vi "MovCorrFuncs 0.1.vi"(7 "Boundary":dbl, 8 "error in (no error)":errorcluster, 9 "MovCorrFunc":T5(ring), 10 "LUT1":cluster{u16, u16}(slide)={0, 4095} caption="Slide" scale=0.0..4095.0, 11 "Image":T3(plugin-control)) -> (0 "error out":errorcluster, 2 "Reference Rectangles":i16[][](array[numeric]), 3 "Reference Screen":T3(plugin-control))   [LabVIEW 2020]
uses:
  <vilib>/vision/Image Controls.llb/IMAQ Image.ctl
panel:
  in  "LUT 2":cluster{i16, i16}(slide)={0, 4095} scale=0.0..4095.0
  in  "LUT":cluster{i16, i16}(slide)={0, 4095} scale=0.0..4095.0
  out "Lines":T1(array[cluster]) {"End Point"."Y" format="%.2f"; "End Point"."X" format="%.2f"; "Start Point"."Y" format="%.2f"; "Start Point"."X" format="%.2f"}
  out "Number of Matches Returned":i32
  out "most Verital":T2
  out "most horizontal":T2
  out "got copy":bool=TRUE
  out "upper":u16
  out "lower":u16
  out "Number of Particles":i32
  out "Mean Value":sgl format="%.2f"
  out "Histogram Graph":T4 {"Incremental Value" format="%.2f"; "Starting Value" format="%.2f"}
  out "temp copy":T3
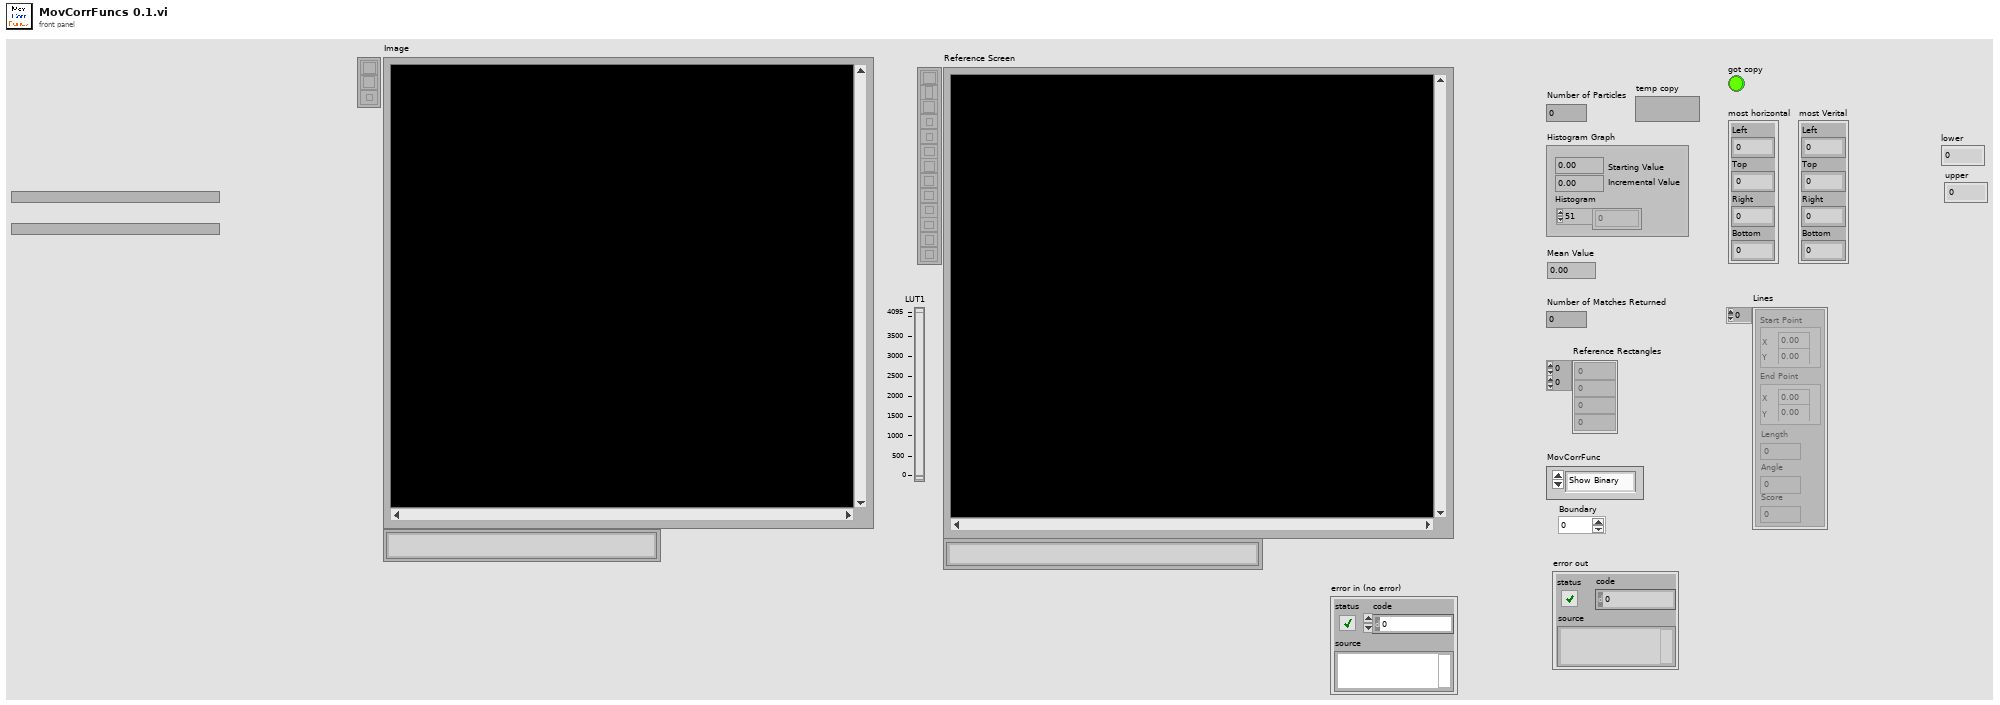
[diagram p1: front panel]
types:
  T1 = cluster{"Start Point":cluster{"X":sgl, "Y":sgl}, "End Point":cluster{"X":sgl, "Y":sgl}, "Length":dbl, "Angle":dbl, "Score":dbl}[]
  T2 = cluster{"Left":i32, "Top":i32, "Right":i32, "Bottom":i32}
  T3 = typedef "IMAQ Image.ctl" = refnum<image>
  T4 = cluster{"Starting Value":sgl, "Incremental Value":sgl, "Histogram":u32[]}
  T5 = enum16{"Show Binary", "Show Dendrite", "Find Lines"}
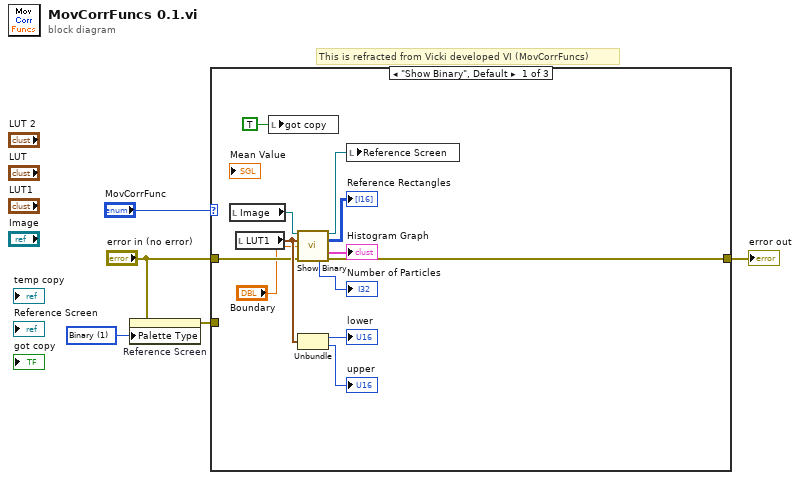
[diagram p0: block diagram]
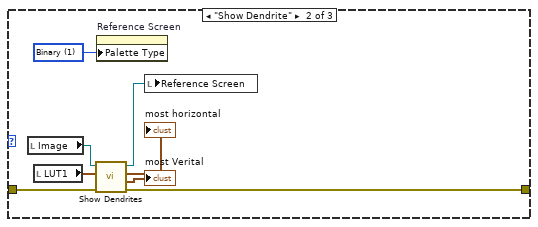
[diagram p2: hidden frame]
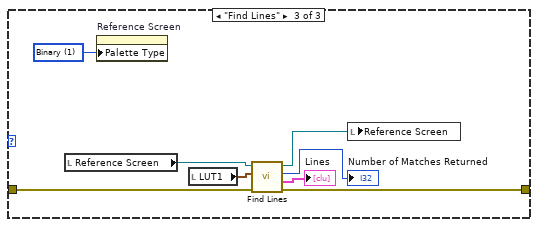
[diagram p3: hidden frame]
diagram:
  w3 = u32 1 items=["Grayscale", "Binary", "Gradient", "Rainbow", "Temperature", "User Defined"] ("Palette:Palette Type")
  # "This is refracted from Vicki developed VI (MovCorrFuncs)"
  n1 = property on="Reference Screen" class="ImageControl"(error in="error in (no error)", "Palette Type"=w3) -> (error out=w1:errorcluster)  [unwired: 1 in, 1 out]
  n2 = case shown="\"Show Binary\", Default" "MovCorrFunc" {
    tunnel: "error in (no error)" -> [w8 w20 w27]
    tunnel: [w7 w19 w26] -> w4
    tunnel: w1 -> [_ _ _]
    frame "Show Binary", Default {
      n3 = local read "Image"() -> (w12:T3)
      n4 = local read "LUT1"() -> (w9:cluster{u16, u16})
      n5 = local write "got copy"(TRUE) -> ()
      n6 = call "Show Binary.vi"("Input Image"=w12, "LUT1"=w9, "Boundary"="Boundary", "error in (no error)"=w8) -> ("Binary Image"=w10:T3, "Reference Rectangles"=→"Reference Rectangles":i16[][], "Histogram Graph"=→"Histogram Graph":T4, "Number of Particles"=→"Number of Particles":i32, "error out"=w7:errorcluster)  [unwired: 7 in]
      n7 = Unbundle(w9) -> (→"lower":u16, →"upper":u16)
      n8 = local write "Reference Screen"(w10) -> ()
    }
    frame "Show Dendrite" {
      w25 = u32 1 items=["Grayscale", "Binary", "Gradient", "Rainbow", "Temperature", "User Defined"] ("Palette:Palette Type")
      n9 = local read "Image"() -> (w24:T3)
      n10 = local read "LUT1"() -> (w21:cluster{u16, u16})
      n11 = call "Show Dendrites.vi"("error in (no error)"=w20, "LUT1"=w21, "Input Image"=w24) -> ("error out"=w19:errorcluster, "most Verital"=→"most Verital":T2, "most horizontal"=→"most horizontal":T2, "Reference Screen"=w23:T3)  [unwired: 3 in, 2 out]
      n12 = property on="Reference Screen" class="ImageControl"("Palette Type"=w25) -> ()  [unwired: 2 in, 2 out]
      n13 = local write "Reference Screen"(w23) -> ()
    }
    frame "Find Lines" {
      w31 = u32 1 items=["Grayscale", "Binary", "Gradient", "Rainbow", "Temperature", "User Defined"] ("Palette:Palette Type")
      n14 = local read "Reference Screen"() -> (w33:T3)
      n15 = property on="Reference Screen" class="ImageControl"("Palette Type"=w31) -> ()  [unwired: 2 in, 2 out]
      n16 = local read "LUT1"() -> (w32:cluster{u16, u16})
      n17 = call "Find Lines.vi"("error in (no error)"=w27, "LUT"=w32, "Image In"=w33) -> ("error out"=w26:errorcluster, "Lines"=→"Lines":T1, "Number of Matches Returned"=→"Number of Matches Returned":i32, "Image Out"=w30:T3)  [unwired: 5 in]
      n18 = local write "Reference Screen"(w30) -> ()
    }
  }
  "error out" <- w4
